vi "AutoCoordinator.vi"(0 "Steps":T3[](array[typedef]) {"ArmPath"."ExtendTrajectory"."Time (ms)" items=["TrajectoryDuration_0ms"=0, "TrajectoryDuration_5ms"=5, "TrajectoryDuration_10ms"=10, "TrajectoryDuration_20ms"=20, "TrajectoryDuration_30ms"=30, "TrajectoryDuration_40ms"=40, "TrajectoryDuration_50ms"=50, "TrajectoryDuration_100ms"=100]; "ArmPath"."RotateTrajectory"."Time (ms)" items=["TrajectoryDuration_0ms"=0, "TrajectoryDuration_5ms"=5, "TrajectoryDuration_10ms"=10, "TrajectoryDuration_20ms"=20, "TrajectoryDuration_30ms"=30, "TrajectoryDuration_40ms"=40, "TrajectoryDuration_50ms"=50, "TrajectoryDuration_100ms"=100]}, 1 "Test":bool, 2 "MotionPlanningNotifiers":T1, 3 "Start":bool, 5 "Stop":bool) -> (6 "IntakeState":T2, 7 "Claw Open":bool, 8 "Done":bool)   [LabVIEW 2017]
uses:
  TypeDef/AutoPreProcessedStep.ctl
  PathPlannerSupport/TypeDefs/DrivePlanResponse.ctl
  Pathfinder/Pathfinder-LabVIEW/Pathfinder-Lib/VIs/Segment.ctl
  Implements/Arm/TypeDefs/ArmPlanResponse.ctl
  General/MotionProfiling/TypeDefs/TrajectoryPoint.ctl
  <vilib>/Rock Robotics/WPI/ThirdParty/Phoenix-LabVIEW/Motor Controller/Controls/CTRE_Phoenix_MotorControl_TrajectoryPointTimeDur.ctl
  TypeDef/AutoWaypointType.ctl
  Implements/Arm/TypeDefs/ArmTargetPosition.ctl
  Implements/TypeDefs/IntakeState.ctl
  TypeDefs/RobotComponents/MotionPlanningNotifiers.ctl
  PathPlannerSupport/TypeDefs/DrivePlanRequest.ctl
  Pathfinder/Pathfinder-LabVIEW/Pathfinder-Lib/VIs/Waypoint.ctl
  Implements/Arm/TypeDefs/ArmPlanRequest.ctl
  ArgosLib/Signal Processing/TypeDefs/EdgeDetector_Type.ctl
  ArgosLib/ArgosLib.lvlib
  Pathfinder/Pathfinder-LabVIEW/Pathfinder-Lib/Pathfinder.lvlib
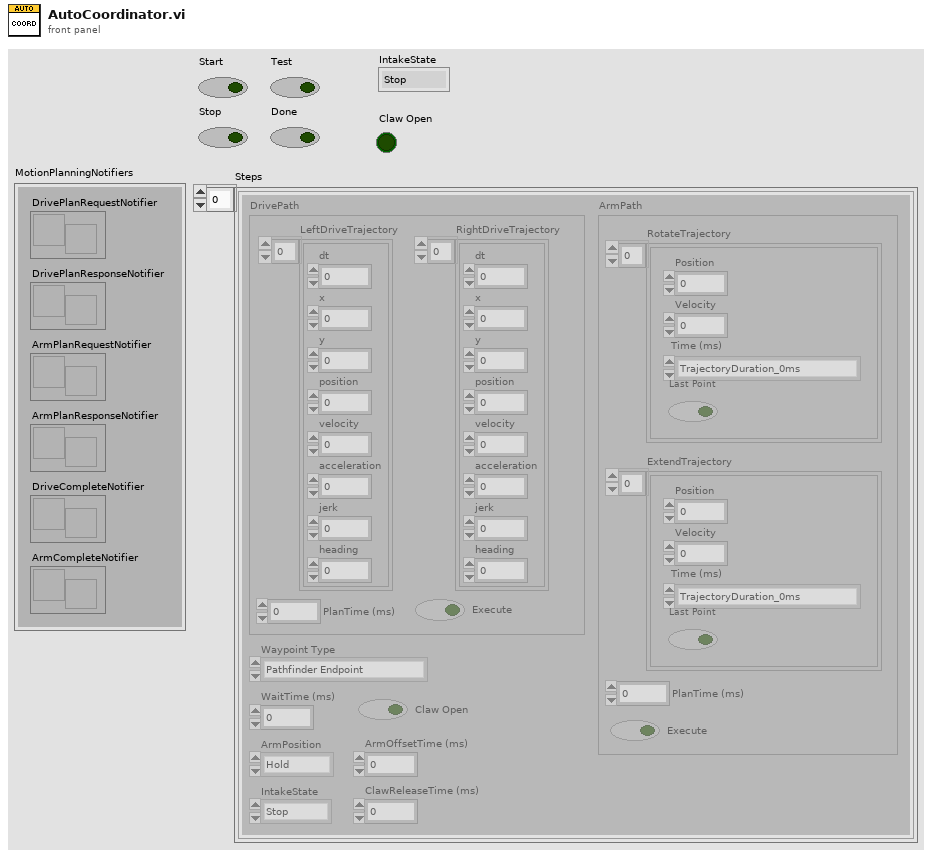
[diagram p1: front panel]
types:
  T1 = typedef "MotionPlanningNotifiers.ctl" = cluster{"DrivePlanRequestNotifier":refnum<notifier>, "DrivePlanResponseNotifier":refnum<notifier>, "ArmPlanRequestNotifier":refnum<notifier>, "ArmPlanResponseNotifier":refnum<notifier>, "DriveCompleteNotifier":refnum<notifier>, "ArmCompleteNotifier":refnum<notifier>}
  T2 = typedef "IntakeState.ctl" = enum16{"Stop", "Forward", "Reverse", "Forward Open"}
  T3 = typedef "AutoPreProcessedStep.ctl" = cluster{"DrivePath":T4, "ArmPath":T6, "Waypoint Type":T9, "WaitTime (ms)":u16, "ArmPosition":T10, "IntakeState":T2, "Claw Open":bool, "ArmOffsetTime (ms)":u16, "ClawReleaseTime (ms)":i32}
  T4 = typedef "DrivePlanResponse.ctl" = cluster{"LeftDriveTrajectory":T5[], "RightDriveTrajectory":T5[], "PlanTime (ms)":u32, "Execute":bool}
  T5 = typedef "Pathfinder.lvlib/Segment.ctl" = cluster{"dt":dbl, "x":dbl, "y":dbl, "position":dbl, "velocity":dbl, "acceleration":dbl, "jerk":dbl, "heading":dbl}
  T6 = typedef "ArmPlanResponse.ctl" = cluster{"RotateTrajectory":T7[], "ExtendTrajectory":T7[], "PlanTime (ms)":u32, "Execute":bool}
  T7 = typedef "TrajectoryPoint.ctl" = cluster{"Position ":dbl, "Velocity ":dbl, "Time (ms)":T8, "Last Point":bool}
  T8 = typedef "CTRE_Phoenix_MotorControl_TrajectoryPointTimeDur.ctl" = i32
  T9 = typedef "AutoWaypointType.ctl" = enum16{"Pathfinder Endpoint", "Pathfinder Waypoint", "Zero-Radius Turn Endpoint", "Stationary", "Vision Assist Endpoint", "Stop"}
  T10 = typedef "ArmTargetPosition.ctl" = enum16{"Hold", "Switch", "Scale Low", "Scale High", "Climb", "Back Place"}
  T11 = typedef "ArgosLib.lvlib/EdgeDetector_Type.ctl" = enum16{"RisingEdge", "FallingEdge", "Both"}
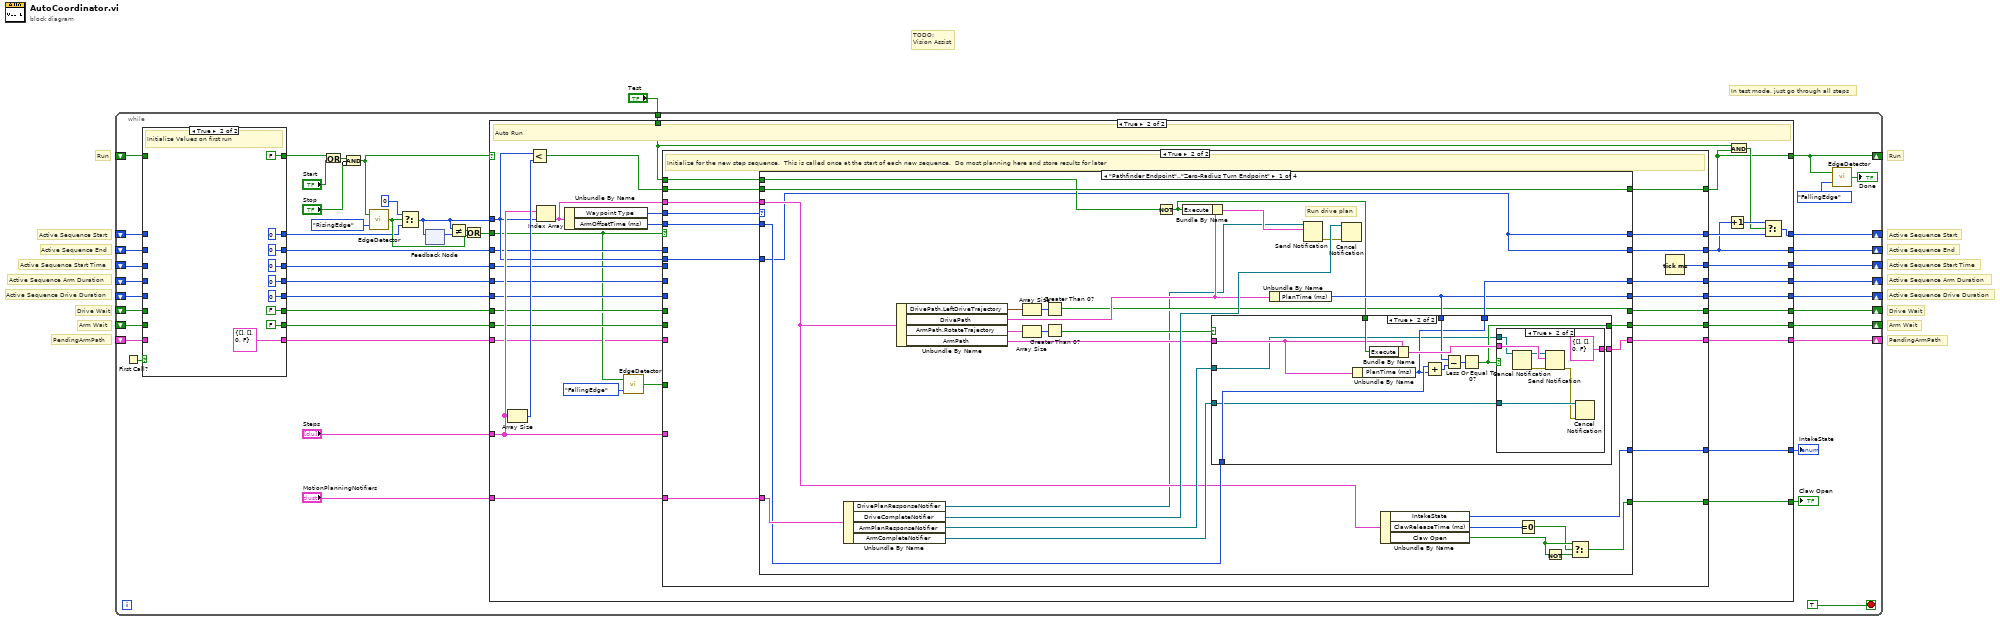
[diagram p0: block diagram]
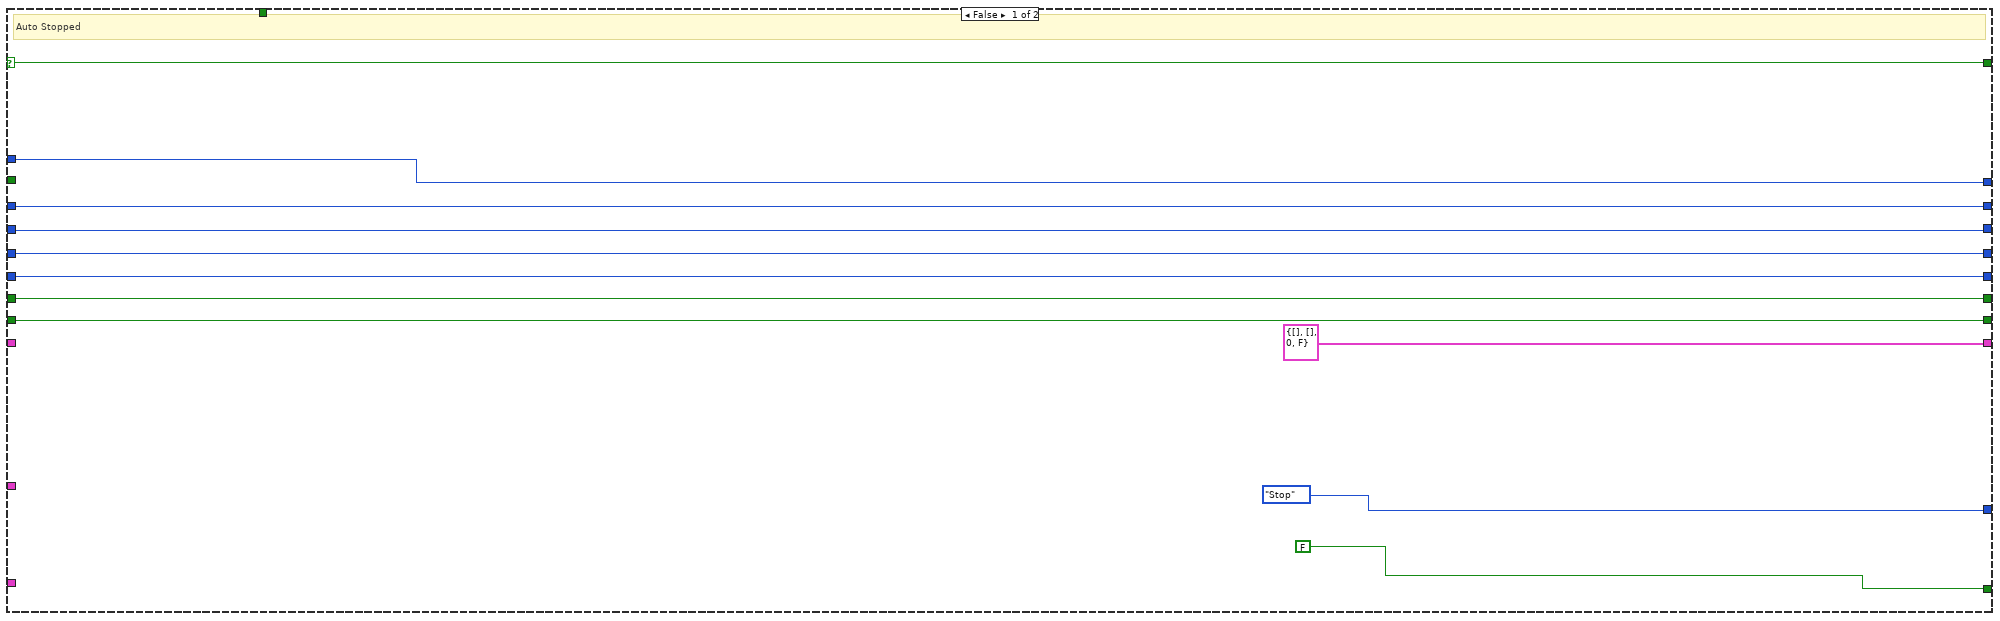
[diagram p3: hidden frame]
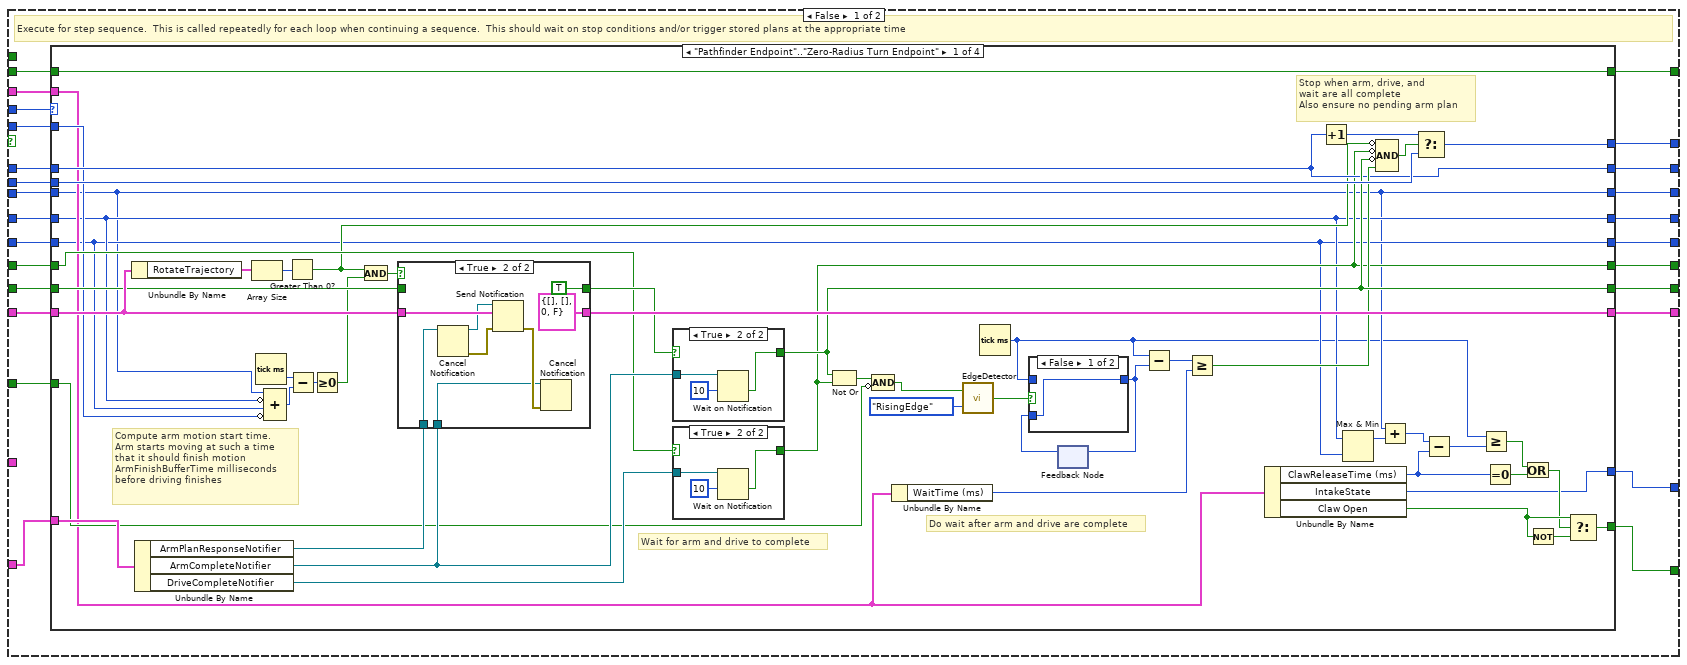
[diagram p4: hidden frame]
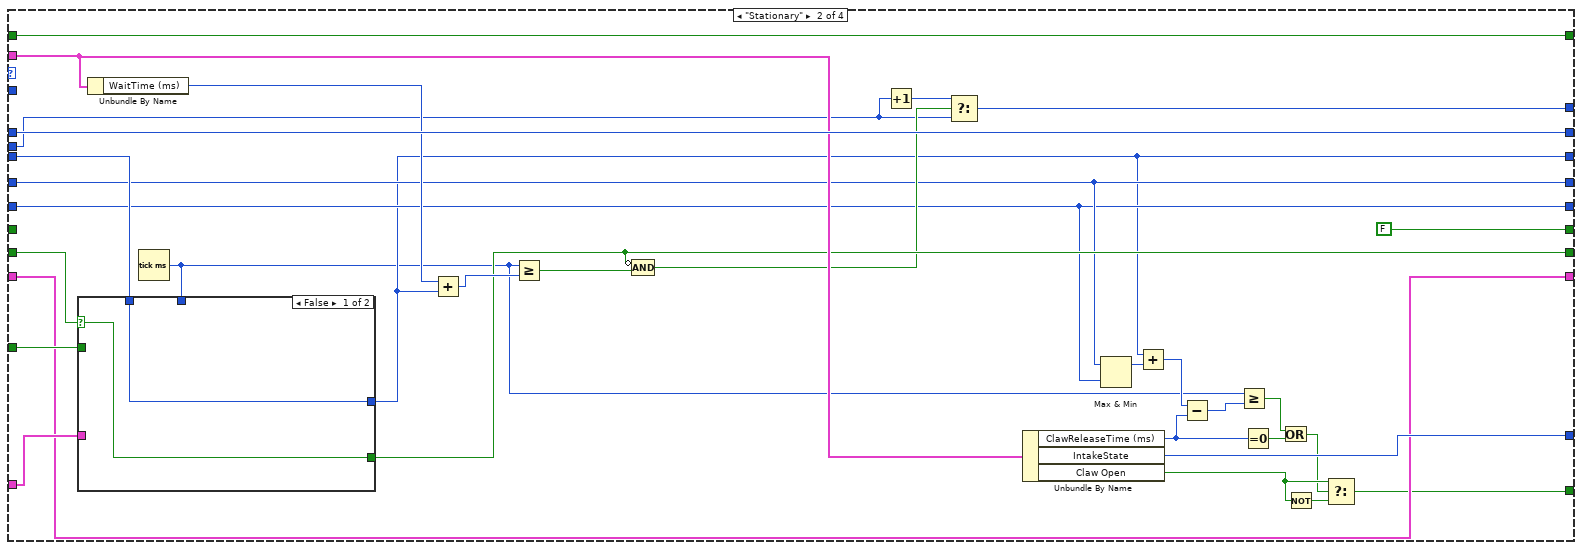
[diagram p9: hidden frame]
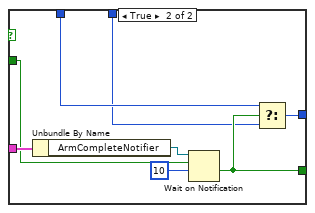
[diagram p10: hidden frame]
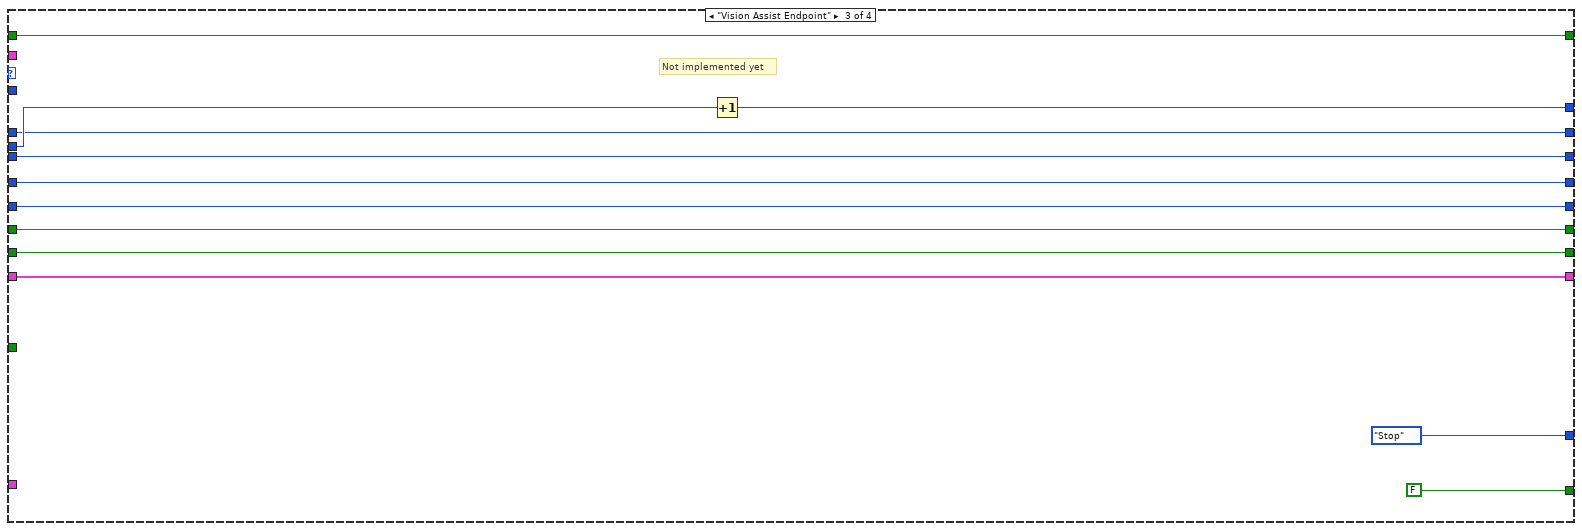
[diagram p11: hidden frame]
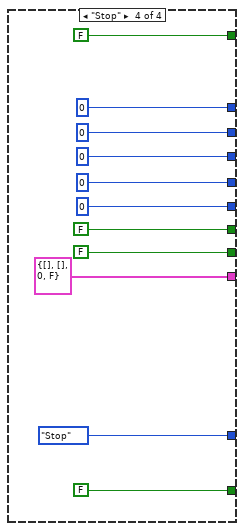
[diagram p12: hidden frame]
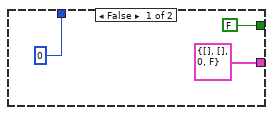
[diagram p13: hidden frame]
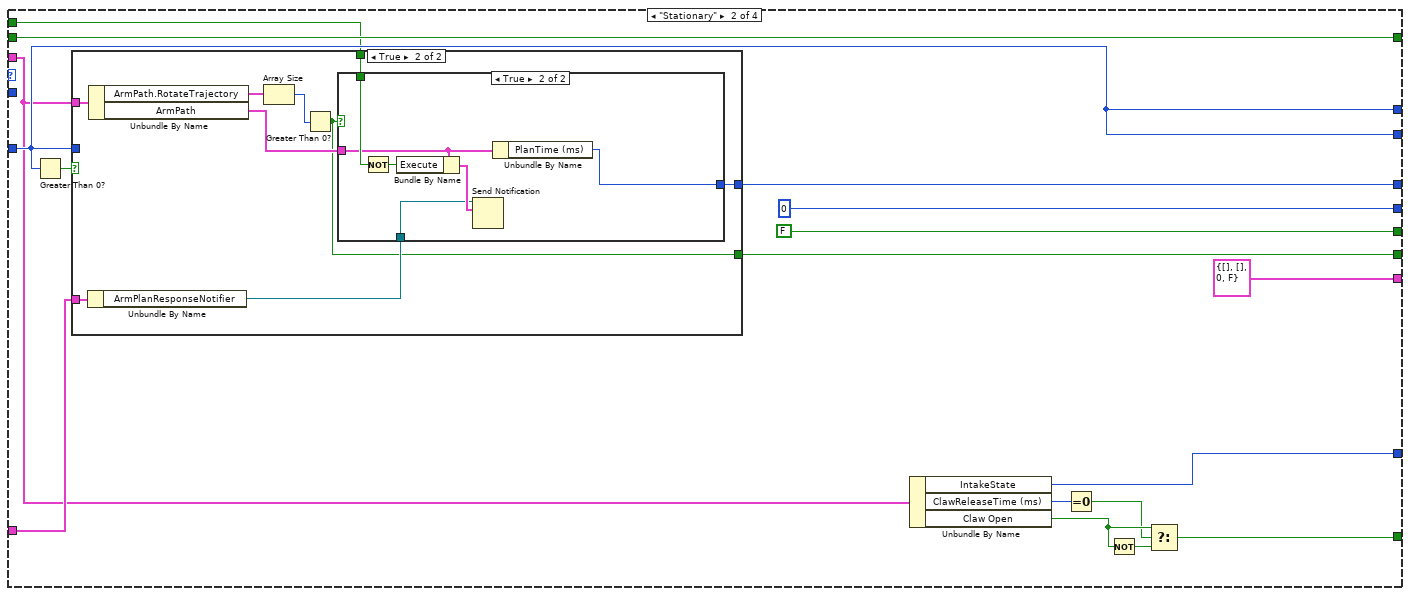
[diagram p15: hidden frame]
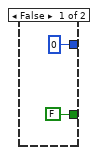
[diagram p16: hidden frame]
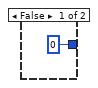
[diagram p17: hidden frame]
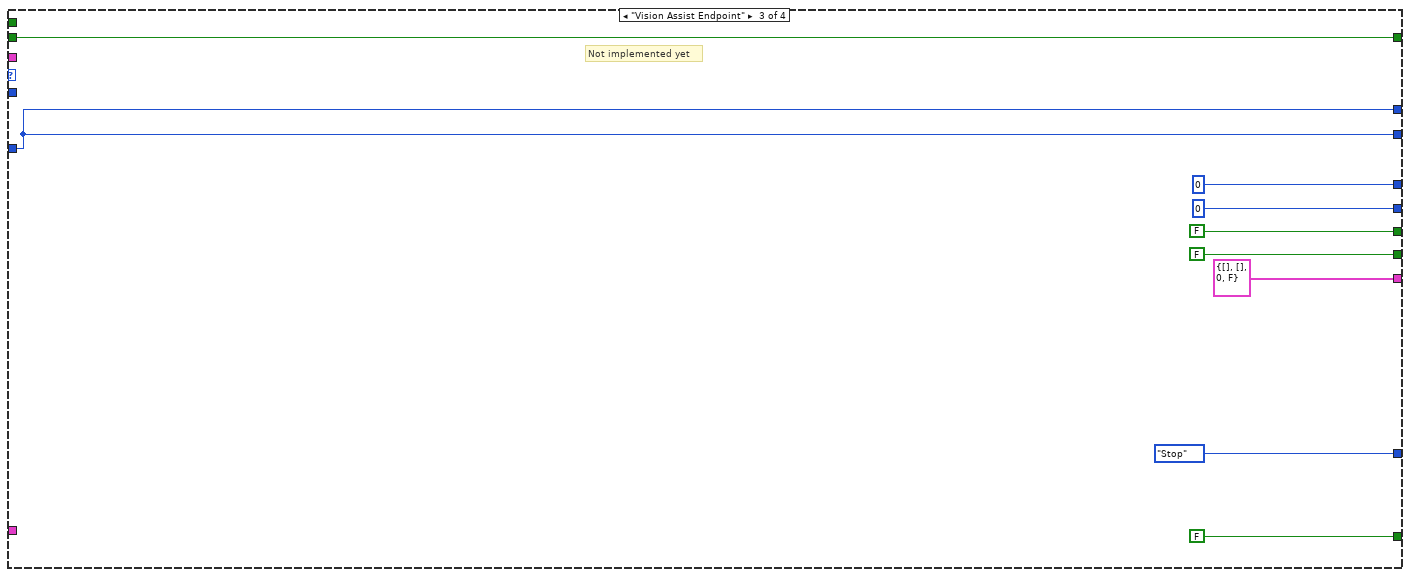
[diagram p18: hidden frame]
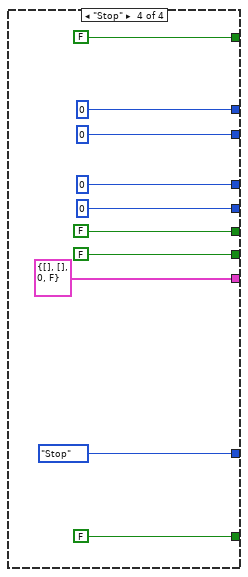
[diagram p19: hidden frame]
diagram:
  # "In test mode, just go through all steps"
  # "PendingArmPath"
  # "PendingArmPath"
  # "TODO:\nVision Assist"
  # "Run"
  # "Arm Wait"
  # "Drive Wait"
  # "Active Sequence Drive Duration"
  # "Active Sequence Arm Duration"
  # "Active Sequence Start Time"
  # "Active Sequence End"
  # "Active Sequence Start"
  # "Arm Wait"
  # "Drive Wait"
  # "Active Sequence Drive Duration"
  # "Active Sequence Arm Duration"
  # "Active Sequence Start Time"
  # "Active Sequence End"
  # "Active Sequence Start"
  # "Run"
  n1 = while {
    shift-right: [w4] -> _
    shift-left: _ -> [w22]
    shift-right: [w41] -> _
    shift-left: _ -> [w20]
    shift-right: [w31] -> _
    shift-left: _ -> [w12]
    shift-right: [w30] -> _
    shift-left: _ -> [w11]
    shift-right: [w26] -> _
    shift-left: _ -> [w10]
    shift-right: [w29] -> _
    shift-left: _ -> [w9]
    shift-right: [w28] -> _
    shift-left: _ -> [w8]
    shift-right: [w27] -> _
    shift-left: _ -> [w7]
    shift-right: [w25] -> _
    shift-left: _ -> [w6]
    tunnel: "Test" -> [w5]
    stop <- TRUE stop-if-true
    n2 = First Call?() -> (First Call?: T/F=w24:bool)
    n3 = case shown="True" w24 {
      tunnel: [w57 FALSE] -> w23
      tunnel: w22 -> [w57 _]
      tunnel: [w56 0] -> w21
      tunnel: w20 -> [w56 _]
      tunnel: [w55 0] -> w19
      tunnel: [w54 u32 0 ("millisecond timer value")] -> w18
      tunnel: [w53 u32 0 ("PlanTime (ms)")] -> w17
      tunnel: [w52 u32 0 ("PlanTime (ms)")] -> w16
      tunnel: [w51 FALSE ("timed out?")] -> w15
      tunnel: [w50 FALSE ("timed out?")] -> w14
      tunnel: [w49 T6 {"RotateTrajectory"=[], "ExtendTrajectory"=[], "PlanTime (ms)"=0, "Execute"=FALSE} ("ArmPlanResponse")] -> w13
      tunnel: w12 -> [w55 _]
      tunnel: w11 -> [w54 _]
      tunnel: w10 -> [w53 _]
      tunnel: w9 -> [w52 _]
      tunnel: w8 -> [w51 _]
      tunnel: w7 -> [w50 _]
      tunnel: w6 -> [w49 _]
      frame False {
      }
      frame True {
        # "Initialize Values on first run"
      }
    }
    n4 = Or(x=w23, y="Start") -> (x .or. y?=w46:bool)
    n5 = Compound Arithmetic op=AND(w46, invert "Stop") -> (w42:bool)
    n6 = call "EdgeDetector.vi"("DetectorType"=EdgeDetector_Type."RisingEdge", "Input"=w42) -> ("Edge"=w33:bool)
    n7 = Select(t=0, s=w33, f=w21) -> (s? t:f=w35:i32)
    n8 = feedback-in #1(w35) -> ()
    n9 = feedback #1() -> (w36:i32)  [unwired: 1 in]
    n10 = Not Equal?(x=w35, y=w36) -> (x != y?=w34:bool)
    n11 = Or(x=w34, y=w33) -> (x .or. y?=w32:bool)
    n12 = case shown="True" w42 {
      selector: w42 -> [w76 _]
      tunnel: [w76 w79] -> w4
      tunnel: w35 -> [w77 w108]
      tunnel: [w77 w83] -> w41
      tunnel: "Steps" -> [_ w109]
      tunnel: [IntakeState."Stop" ("IntakeState") w104] -> w39
      tunnel: [FALSE ("Claw Open") w103] -> w38
      tunnel: "MotionPlanningNotifiers" -> [_ w100]
      tunnel: w32 -> [_ w91]
      tunnel: [w73 w81] -> w31
      tunnel: [w72 w107] -> w30
      tunnel: w18 -> [w72 w106]
      tunnel: [w70 w105] -> w29
      tunnel: [w69 w102] -> w28
      tunnel: [w68 w101] -> w27
      tunnel: [w71 w99] -> w26
      tunnel: w19 -> [w73 w92]
      tunnel: w17 -> [w71 w93]
      tunnel: w16 -> [w70 w94]
      tunnel: w15 -> [w69 w96]
      tunnel: w14 -> [w68 w95]
      tunnel: [T6 {"RotateTrajectory"=[], "ExtendTrajectory"=[], "PlanTime (ms)"=0, "Execute"=FALSE} ("ArmPlanResponse") w88] -> w25
      tunnel: w13 -> [_ w87]
      tunnel: w5 -> [_ w78]
      frame False {
        # "Auto Stopped"
      }
      frame True {
        # "Auto Run"
        n13 = Array Size(array=w109) -> (size(s)=w110:i32)
        n14 = Less?(x=w108, y=w110) -> (x < y?=w86:bool)
        n15 = Index Array(array=w109, index=w108) -> (element=w97:T3)
        n16 = Unbundle By Name(w97) -> ("Waypoint Type"=w98:T9, "ArmOffsetTime (ms)"=w85:u16)
        n17 = call "EdgeDetector.vi"("DetectorType"=EdgeDetector_Type."FallingEdge", "Input"=w91) -> ("Edge"=w89:bool)
        n18 = case shown="True" w91 {
          tunnel: w109 -> [_ _]
          tunnel: w108 -> [w127 w290]
          tunnel: [w126 w289] -> w84
          tunnel: [w125 w288] -> w81
          tunnel: [w116 w287] -> w107
          tunnel: w106 -> [w117 _]
          tunnel: [w123 w286] -> w105
          tunnel: [w120 w285] -> w104
          tunnel: [w119 w284] -> w103
          tunnel: [w122 w283] -> w102
          tunnel: [w121 w282] -> w101
          tunnel: w100 -> [w132 w281]
          tunnel: [w124 w280] -> w99
          tunnel: w98 -> [w135 w279]
          tunnel: w97 -> [w133 w278]
          tunnel: w96 -> [w131 _]
          tunnel: w95 -> [w130 _]
          tunnel: w94 -> [w129 _]
          tunnel: w93 -> [w128 _]
          tunnel: w92 -> [w134 _]
          tunnel: w89 -> [w118 _]
          tunnel: [w115 w277] -> w88
          tunnel: w87 -> [w114 _]
          tunnel: w86 -> [w113 w276]
          tunnel: [w112 w275] -> w79
          tunnel: w85 -> [w111 w274]
          tunnel: w78 -> [_ w273]
          frame False {
            # "Execute for step sequence.  This is called repeatedly for each loop when continuing a sequence.  This should wait on stop conditions and/or trigger stored plans at the appropriate time"
            n19 = case shown="\"Pathfinder Endpoint\"..\"Zero-Radius Turn Endpoint\"" w135 {
              tunnel: w134 -> [w158 w234 w255 _]
              tunnel: w133 -> [w140 w233 _ _]
              tunnel: w132 -> [w181 w237 _ _]
              tunnel: w131 -> [w157 _ w259 _]
              tunnel: w130 -> [w177 w239 w258 _]
              tunnel: w129 -> [w138 w215 w260 _]
              tunnel: w128 -> [w139 w216 w261 _]
              tunnel: w117 -> [w137 w232 w252 _]
              tunnel: w127 -> [w185 w224 w257 _]
              tunnel: [w187 w229 w256 0] -> w126
              tunnel: [w158 w234 w255 0] -> w125
              tunnel: [w139 w216 w261 u32 0 ("PlanTime (ms)")] -> w124
              tunnel: [w138 w215 w260 u32 0 ("PlanTime (ms)")] -> w123
              tunnel: [w155 FALSE w259 FALSE ("timed out?")] -> w122
              tunnel: [w169 w227 w258 FALSE ("timed out?")] -> w121
              tunnel: [w141 w238 IntakeState."Stop" ("IntakeState") IntakeState."Stop" ("IntakeState")] -> w120
              tunnel: [w142 w221 FALSE ("Claw Open") FALSE ("Claw Open")] -> w119
              tunnel: w118 -> [w167 w236 _ _]
              tunnel: [w137 w210 w252 u32 0 ("millisecond timer value")] -> w116
              tunnel: [w178 w223 w251 T6 {"RotateTrajectory"=[], "ExtendTrajectory"=[], "PlanTime (ms)"=0, "Execute"=FALSE} ("ArmPlanResponse")] -> w115
              tunnel: w114 -> [w179 w223 w251 _]
              tunnel: w113 -> [w153 w222 w250 _]
              tunnel: [w153 w222 w250 FALSE] -> w112
              tunnel: w111 -> [w152 _ _ _]
              frame "Pathfinder Endpoint".."Zero-Radius Turn Endpoint" {
                # "Do wait after arm and drive are complete"
                # "Wait for arm and drive to complete"
                # "Stop when arm, drive, and\nwait are all complete\nAlso ensure no pending arm plan"
                # "Compute arm motion start time.\nArm starts moving at such a time\nthat it should finish motion\nArmFinishBufferTime milliseconds\nbefore driving finishes"
                n20 = Unbundle By Name(w179) -> ("RotateTrajectory"=w184:T7[])
                n21 = Unbundle By Name(w181) -> ("ArmPlanResponseNotifier"=w180:refnum<notifier>, "ArmCompleteNotifier"=w171:refnum<notifier>, "DriveCompleteNotifier"=w172:refnum<notifier>)
                n22 = Array Size(array=w184) -> (size(s)=w183:i32)
                n23 = Tick Count (ms)() -> (millisecond timer value=w182:u32)
                n24 = Compound Arithmetic op=ADD(w137, invert w139, w138, invert w152) -> (w154:u32)
                n25 = Greater Than 0?(x=w183) -> (x > 0?=w156:bool)
                n26 = Subtract(x=w182, y=w154) -> (x-y=w175:i32)
                n27 = Greater Or Equal To 0?(x=w175) -> (x >= 0?=w174:bool)
                n28 = And(x=w156, y=w174) -> (x .and. y?=w176:bool)
                n29 = case shown="True" w176 {
                  tunnel: [w198 TRUE] -> w170
                  tunnel: w180 -> [_ w202]
                  tunnel: w179 -> [w199 w205]
                  tunnel: w171 -> [_ w204]
                  tunnel: [w199 T6 {"RotateTrajectory"=[], "ExtendTrajectory"=[], "PlanTime (ms)"=0, "Execute"=FALSE} ("ArmPlanResponse")] -> w178
                  tunnel: w177 -> [w198 _]
                  frame False {
                  }
                  frame True {
                    n30 = Cancel Notification(0:w202) -> (8:w201:refnum<notifier>, 11:w200:errorcluster)  [unwired: 1 in, 1 out]
                    n31 = Send Notification(notification=w205, notifier=w201, error in (no error)=w200) -> (error out=w206:errorcluster)  [unwired: 1 out]
                    n32 = Cancel Notification(0:w204, 3:w206) -> ()  [unwired: 3 out]
                  }
                }
                n33 = case shown="True" w170 {
                  selector: w170 -> [w194 _]
                  tunnel: w171 -> [_ w196]
                  tunnel: [w194 w195] -> w169
                  frame False {
                  }
                  frame True {
                    n34 = Wait on Notification(notifier=w196, timeout in ms (-1)=10) -> (timed out?=w195:bool)  [unwired: 2 in, 3 out]
                  }
                }
                n35 = case shown="True" w157 {
                  selector: w157 -> [w190 _]
                  tunnel: w172 -> [_ w192]
                  tunnel: [w190 w191] -> w155
                  frame False {
                  }
                  frame True {
                    n36 = Wait on Notification(notifier=w192, timeout in ms (-1)=10) -> (timed out?=w191:bool)  [unwired: 2 in, 3 out]
                  }
                }
                n37 = Not Or(1:w155, 2:w169) -> (0:w168:bool)
                n38 = Compound Arithmetic op=AND(w168, invert w167) -> (w165:bool)
                n39 = Unbundle By Name(w140) -> ("WaitTime (ms)"=w160:u16)
                n40 = call "EdgeDetector.vi"("DetectorType"=EdgeDetector_Type."RisingEdge", "Input"=w165) -> ("Edge"=w164:bool)
                n41 = Tick Count (ms)() -> (millisecond timer value=w136:u32)
                n42 = feedback #2() -> (w163:u32)  [unwired: 1 in]
                n43 = case shown="False" w164 {
                  tunnel: w136 -> [_ w189]
                  tunnel: [w188 w189] -> w162
                  tunnel: w163 -> [w188 _]
                  frame False {
                  }
                  frame True {
                  }
                }
                n44 = feedback-in #2(w162) -> ()
                n45 = Subtract(x=w136, y=w162) -> (x-y=w161:u32)
                n46 = Greater Or Equal?(x=w161, y=w160) -> (x >= y?=w159:bool)
                n47 = Unbundle By Name(w140) -> ("ClawReleaseTime (ms)"=w147:i32, "IntakeState"=w141:T2, "Claw Open"=w150:bool)
                n48 = Increment(x=w158) -> (x+1=w186:i32)
                n49 = Max & Min(x=w139, y=w138) -> (max(x,y)=w144:u32)  [unwired: 1 out]
                n50 = Compound Arithmetic op=AND(invert w156, invert w155, invert w169, w159) -> (w173:bool)
                n51 = Add(x=w137, y=w144) -> (x+y=w145:u32)
                n52 = Select(t=w186, s=w173, f=w185) -> (s? t:f=w187:i32)
                n53 = Subtract(x=w145, y=w147) -> (x-y=w143:u32)
                n54 = Greater Or Equal?(x=w136, y=w143) -> (x >= y?=w146:bool)
                n55 = Equal To 0?(x=w147) -> (x = 0?=w149:bool)
                n56 = Or(x=w146, y=w149) -> (x .or. y?=w148:bool)
                n57 = Not(x=w150) -> (.not. x?=w151:bool)
                n58 = Select(t=w150, s=w148, f=w151) -> (s? t:f=w142:bool)
              }
              frame "Stationary" {
                n59 = Unbundle By Name(w233) -> ("WaitTime (ms)"=w230:u16)
                n60 = Tick Count (ms)() -> (millisecond timer value=w208:u32)
                n61 = case shown="False" w239 {
                  selector: w239 -> [w241 _]
                  tunnel: w237 -> [_ w249]
                  tunnel: w236 -> [_ w246]
                  tunnel: [w241 w245] -> w227
                  tunnel: w232 -> [w240 w244]
                  tunnel: w208 -> [_ w243]
                  tunnel: [w240 w242] -> w210
                  frame False {
                  }
                  frame True {
                    n62 = Unbundle By Name(w249) -> ("ArmCompleteNotifier"=w248:refnum<notifier>)
                    n63 = Wait on Notification(notifier=w248, ignore previous (F)=w246, timeout in ms (-1)=10) -> (timed out?=w245:bool)  [unwired: 1 in, 3 out]
                    n64 = Select(t=w244, s=w245, f=w243) -> (s? t:f=w242:u32)
                  }
                }
                n65 = Add(x=w230, y=w210) -> (x+y=w231:u32)
                n66 = Greater Or Equal?(x=w208, y=w231) -> (x >= y?=w228:bool)
                n67 = Compound Arithmetic op=AND(invert w227, w228) -> (w226:bool)
                n68 = Increment(x=w224) -> (x+1=w225:i32)
                n69 = Select(t=w225, s=w226, f=w224) -> (s? t:f=w229:i32)
                n70 = Unbundle By Name(w233) -> ("ClawReleaseTime (ms)"=w214:i32, "IntakeState"=w238:T2, "Claw Open"=w219:bool)
                n71 = Max & Min(x=w216, y=w215) -> (max(x,y)=w211:u32)  [unwired: 1 out]
                n72 = Add(x=w210, y=w211) -> (x+y=w212:u32)
                n73 = Subtract(x=w212, y=w214) -> (x-y=w209:u32)
                n74 = Greater Or Equal?(x=w208, y=w209) -> (x >= y?=w213:bool)
                n75 = Equal To 0?(x=w214) -> (x = 0?=w218:bool)
                n76 = Or(x=w213, y=w218) -> (x .or. y?=w217:bool)
                n77 = Not(x=w219) -> (.not. x?=w220:bool)
                n78 = Select(t=w219, s=w217, f=w220) -> (s? t:f=w221:bool)
              }
              frame "Vision Assist Endpoint" {
                # "Not implemented yet"
                n79 = Increment(x=w257) -> (x+1=w256:i32)
              }
              frame "Stop" {
              }
            }
          }
          frame True {
            # "Initialize for the new step sequence.  This is called once at the start of each new sequence.  Do most planning here and store results for later"
            n80 = case shown="\"Pathfinder Endpoint\"..\"Zero-Radius Turn Endpoint\"" w279 {
              tunnel: w290 -> [w300 w355 w388 _]
              tunnel: w278 -> [w307 w348 _ _]
              tunnel: [w300 w355 w388 0] -> w289
              tunnel: [w300 w355 w388 0] -> w288
              tunnel: [w314 u16 0 u32 0 ("PlanTime (ms)") u32 0 ("PlanTime (ms)")] -> w286
              tunnel: [w303 w347 IntakeState."Stop" ("IntakeState") IntakeState."Stop" ("IntakeState")] -> w285
              tunnel: [w306 w346 FALSE ("Claw Open") FALSE ("Claw Open")] -> w284
              tunnel: [w292 FALSE FALSE FALSE] -> w283
              tunnel: [w312 w358 FALSE FALSE] -> w282
              tunnel: w281 -> [w316 w357 _ _]
              tunnel: [w315 w356 u32 0 ("PlanTime (ms)") u32 0 ("PlanTime (ms)")] -> w280
              tunnel: [w313 T6 {"RotateTrajectory"=[], "ExtendTrajectory"=[], "PlanTime (ms)"=0, "Execute"=FALSE} ("ArmPlanResponse") T6 {"RotateTrajectory"=[], "ExtendTrajectory"=[], "PlanTime (ms)"=0, "Execute"=FALSE} ("ArmPlanResponse") T6 {"RotateTrajectory"=[], "ExtendTrajectory"=[], "PlanTime (ms)"=0, "Execute"=FALSE} ("ArmPlanResponse")] -> w277
              tunnel: w276 -> [w311 w353 w380 _]
              tunnel: [w311 w353 w380 FALSE] -> w275
              tunnel: w274 -> [w310 _ _ _]
              tunnel: w273 -> [w302 w345 _ _]
              frame "Pathfinder Endpoint".."Zero-Radius Turn Endpoint" {
                # "Run drive plan"
                n81 = Unbundle By Name(w316) -> ("DrivePlanResponseNotifier"=w291:refnum<notifier>, "DriveCompleteNotifier"=w320:refnum<notifier>, "ArmPlanResponseNotifier"=w321:refnum<notifier>, "ArmCompleteNotifier"=w319:refnum<notifier>)
                n82 = Unbundle By Name(w307) -> ("DrivePath.LeftDriveTrajectory"=w294:T5[], "DrivePath"=w295:T4, "ArmPath.RotateTrajectory"=w299:T7[], "ArmPath"=w296:T6)
                n83 = Array Size(array=w294) -> (size(s)=w293:i32)
                n84 = Array Size(array=w299) -> (size(s)=w298:i32)
                n85 = Greater Than 0?(x=w293) -> (x > 0?=w292:bool)
                n86 = Greater Than 0?(x=w298) -> (x > 0?=w297:bool)
                n87 = Not(x=w302) -> (.not. x?=w301:bool)
                n88 = Bundle By Name(cluster=w295, "Execute"=w301) -> (w317:T4)
                n89 = Unbundle By Name(w295) -> ("PlanTime (ms)"=w314:u32)
                n90 = case shown="True" w297 {
                  tunnel: w321 -> [_ w325]
                  tunnel: [T6 {"RotateTrajectory"=[], "ExtendTrajectory"=[], "PlanTime (ms)"=0, "Execute"=FALSE} ("ArmPlanResponse") w331] -> w313
                  tunnel: [u32 0 ("PlanTime (ms)") w328] -> w315
                  tunnel: w319 -> [_ w330]
                  tunnel: w310 -> [_ w336]
                  tunnel: w314 -> [_ w329]
                  tunnel: [FALSE w332] -> w312
                  tunnel: w301 -> [_ w327]
                  tunnel: w296 -> [_ w326]
                  frame False {
                  }
                  frame True {
                    n91 = Unbundle By Name(w326) -> ("PlanTime (ms)"=w328:u32)
                    n92 = Bundle By Name(cluster=w326, "Execute"=w327) -> (w333:T6)
                    n93 = Add(x=w336, y=w328) -> (x+y=w335:u32)
                    n94 = Subtract(x=w329, y=w335) -> (x-y=w334:i32)
                    n95 = Less Or Equal To 0?(x=w334) -> (x <= 0?=w332:bool)
                    n96 = case shown="True" w332 {
                      tunnel: w333 -> [w337 w344]
                      tunnel: [w337 T6 {"RotateTrajectory"=[], "ExtendTrajectory"=[], "PlanTime (ms)"=0, "Execute"=FALSE} ("ArmPlanResponse")] -> w331
                      tunnel: w325 -> [_ w339]
                      tunnel: w330 -> [_ w343]
                      frame False {
                      }
                      frame True {
                        n97 = Cancel Notification(0:w339) -> (8:w338:refnum<notifier>, 11:w340:errorcluster)  [unwired: 1 in, 1 out]
                        n98 = Send Notification(notification=w344, notifier=w338, error in (no error)=w340) -> (error out=w341:errorcluster)  [unwired: 1 out]
                        n99 = Cancel Notification(0:w343, 3:w341) -> ()  [unwired: 3 out]
                      }
                    }
                  }
                }
                n100 = Send Notification(notification=w317, notifier=w291) -> (error out=w318:errorcluster)  [unwired: 1 in, 1 out]
                n101 = Cancel Notification(0:w320, 3:w318) -> ()  [unwired: 3 out]
                n102 = Unbundle By Name(w307) -> ("IntakeState"=w303:T2, "ClawReleaseTime (ms)"=w304:i32, "Claw Open"=w308:bool)
                n103 = Equal To 0?(x=w304) -> (x = 0?=w305:bool)
                n104 = Not(x=w308) -> (.not. x?=w309:bool)
                n105 = Select(t=w308, s=w305, f=w309) -> (s? t:f=w306:bool)
              }
              frame "Stationary" {
                n106 = Greater Than 0?(x=w355) -> (x > 0?=w359:bool)
                n107 = case shown="True" w359 {
                  tunnel: w355 -> [_ _]
                  tunnel: w348 -> [_ w369]
                  tunnel: [FALSE w364] -> w358
                  tunnel: w357 -> [_ w372]
                  tunnel: [u32 0 ("PlanTime (ms)") w371] -> w356
                  tunnel: w345 -> [_ w370]
                  frame False {
                  }
                  frame True {
                    n108 = Unbundle By Name(w372) -> ("ArmPlanResponseNotifier"=w368:refnum<notifier>)
                    n109 = Unbundle By Name(w369) -> ("ArmPath.RotateTrajectory"=w366:T7[], "ArmPath"=w367:T6)
                    n110 = Array Size(array=w366) -> (size(s)=w365:i32)
                    n111 = Greater Than 0?(x=w365) -> (x > 0?=w364:bool)
                    n112 = case shown="True" w364 {
                      tunnel: [u32 0 ("PlanTime (ms)") w374] -> w371
                      tunnel: w370 -> [_ w376]
                      tunnel: w368 -> [_ w378]
                      tunnel: w367 -> [_ w375]
                      frame False {
                      }
                      frame True {
                        n113 = Not(x=w376) -> (.not. x?=w377:bool)
                        n114 = Bundle By Name(cluster=w375, "Execute"=w377) -> (w379:T6)
                        n115 = Send Notification(notification=w379, notifier=w378) -> ()  [unwired: 1 in, 2 out]
                        n116 = Unbundle By Name(w375) -> ("PlanTime (ms)"=w374:u32)
                      }
                    }
                  }
                }
                n117 = Unbundle By Name(w348) -> ("IntakeState"=w347:T2, "ClawReleaseTime (ms)"=w352:i32, "Claw Open"=w350:bool)
                n118 = Equal To 0?(x=w352) -> (x = 0?=w349:bool)
                n119 = Not(x=w350) -> (.not. x?=w351:bool)
                n120 = Select(t=w350, s=w349, f=w351) -> (s? t:f=w346:bool)
              }
              frame "Vision Assist Endpoint" {
                # "Not implemented yet"
              }
              frame "Stop" {
              }
            }
            n121 = Tick Count (ms)() -> (millisecond timer value=w287:u32)
          }
        }
        n122 = Increment(x=w81) -> (x+1=w82:i32)
        n123 = And(x=w78, y=w79) -> (x .and. y?=w80:bool)
        n124 = Select(t=w82, s=w80, f=w84) -> (s? t:f=w83:i32)
      }
    }
    "IntakeState" <- w39
    "Claw Open" <- w38
    n125 = call "EdgeDetector.vi"("DetectorType"=EdgeDetector_Type."FallingEdge", "Input"=w4) -> ("Edge"=→"Done":bool)
  }
